vi "列表消息json处理.vi"(6 "error in (no error)":errorcluster caption="错误输入（无错误）", 7 "json input":string) -> (0 "error out":errorcluster caption="错误输出", 1 "top_stories":T1(array[cluster]), 2 "stories":T1(array[cluster]), 3 "date":string)   [LabVIEW 2012]
uses:
  <vilib>/addons/JSON API/JSON Value/JSON Value.lvclass
  <vilib>/addons/JSON API/JSON Value/Set from JSON string.vi
  <vilib>/addons/JSON API/Get Polymorphic/JSON GetSet.lvlib
  <vilib>/addons/JSON API/JSON Scalar/JSON Scalar.lvclass
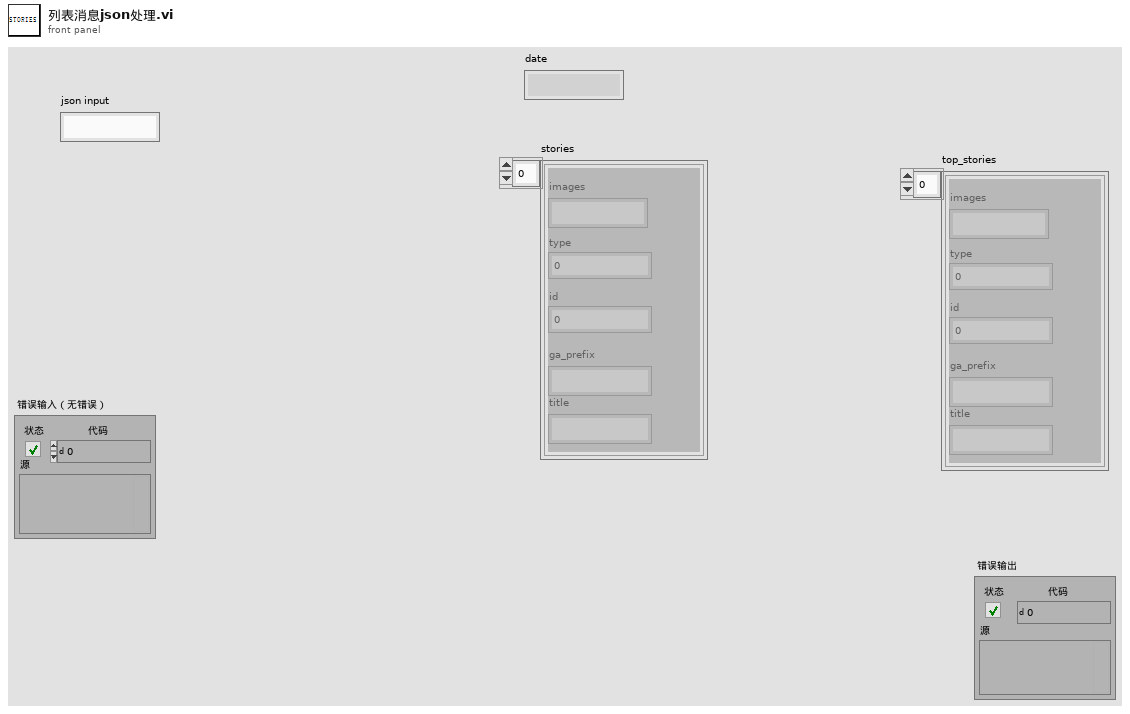
[diagram p1: front panel]
types:
  T1 = cluster{"images":string, "type":i32, "id":i64, "ga_prefix":string, "title":string}[]
  T2 = cluster{"LabVIEW Text":string, "Number":i32, "Number":i32, "LabVIEW Text":string, "LabVIEW Text":string}
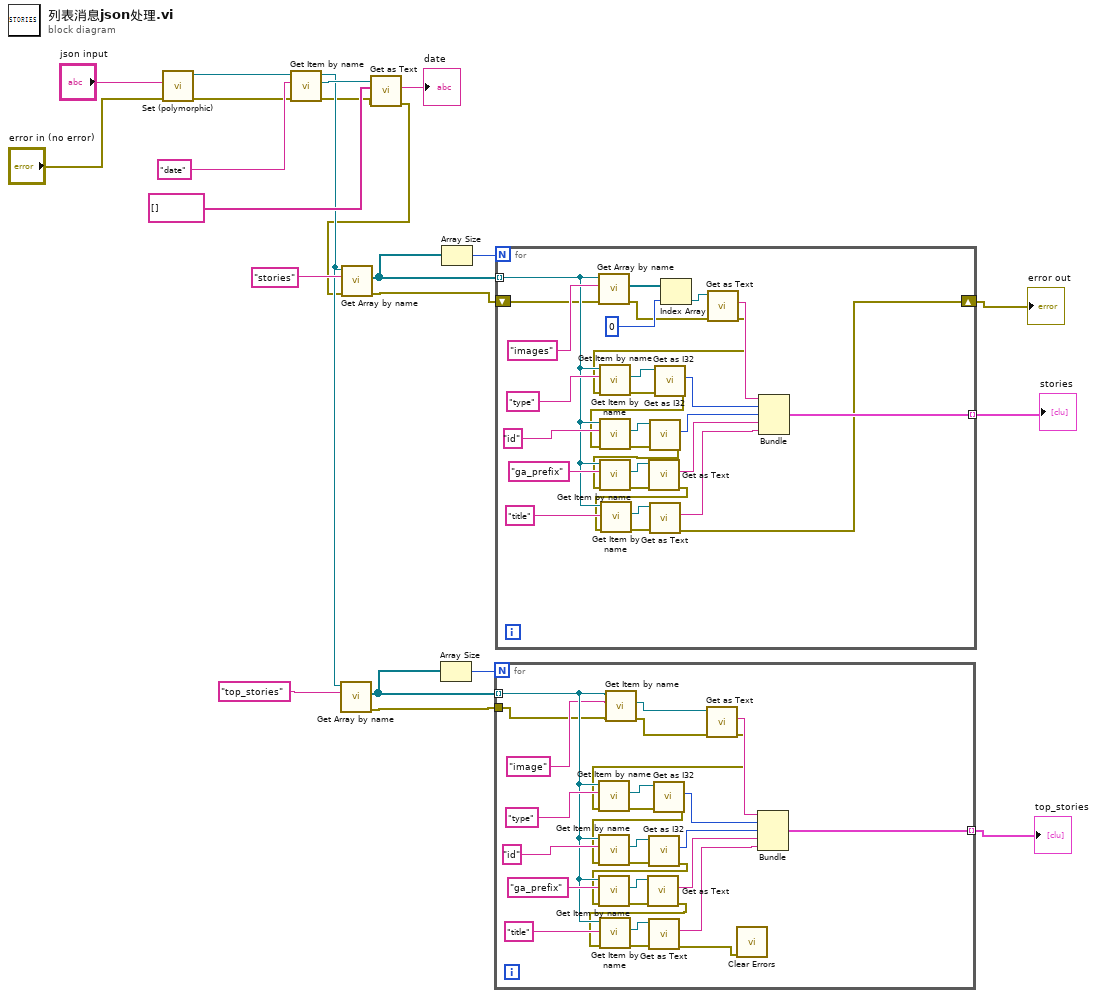
[diagram p0: block diagram]
diagram:
  n1 = call-poly <vilib>:"Set (polymorphic).vi"("error in (no error)"="error in (no error)", "JSON stream"="json input") -> ("error out"=w20:errorcluster, "JSON Value out"=w22:refnum<class "JSON Value.lvclass">)  [unwired: 7 in, 1 out]
  n2 = call-dynamic "Get Item by name.vi"("error in (no error)"=w20, "name"="date", "JSON Value In"=w22) -> ("error out"=w3:errorcluster, "Value"=w19:refnum<class "JSON Value.lvclass">, "JSON Value Out"=w6:refnum<class "JSON Value.lvclass">)  [unwired: 5 in, 1 out]
  n3 = call <vilib>:"Get Array by name.vi"("name"="top_stories", "JSON Value In"=w6) -> ("error out"=w7:errorcluster, "Array"=w8:refnum<class "JSON Value.lvclass">[])  [unwired: 6 in, 2 out]
  n4 = call <vilib>:"Get as Text.vi"("error in (no error)"=w3, "Name Array"=string[] [], "JSON Scalar in"=w19) -> ("error out"=w2:errorcluster, "LabVIEW Text"=→"date":string)  [unwired: 6 in, 1 out]
  n5 = call <vilib>:"Get Array by name.vi"("error in (no error)"=w2, "name"="stories", "JSON Value In"=w6) -> ("error out"=w12:errorcluster, "Array"=w13:refnum<class "JSON Value.lvclass">[])  [unwired: 5 in, 2 out]
  n6 = Array Size(array=w8) -> (size(s)=w9:i32)
  n7 = Array Size(array=w13) -> (size(s)=w14:i32)
  n8 = for {
    N: w9 -> [_]
    tunnel: w8 -> [w32] mode=indexing
    tunnel: w7 -> [w30]
    tunnel: [w33] -> w5 mode=indexing
    n9 = call-dynamic "Get Item by name.vi"("error in (no error)"=w30, "name"="image", "JSON Value In"=w32) -> ("error out"=w28:errorcluster, "Value"=w29:refnum<class "JSON Value.lvclass">)  [unwired: 5 in, 2 out]
    n10 = call <vilib>:"Get as Text.vi"("error in (no error)"=w28, "JSON Scalar in"=w29) -> ("error out"=w27:errorcluster, "LabVIEW Text"=w38:string)  [unwired: 7 in, 1 out]
    n11 = call-dynamic "Get Item by name.vi"("error in (no error)"=w27, "name"="type", "JSON Value In"=w32) -> ("error out"=w45:errorcluster, "Value"=w49:refnum<class "JSON Value.lvclass">)  [unwired: 5 in, 2 out]
    n12 = call <vilib>:"Get as I32.vi"("error in (no error)"=w45, "JSON Scalar in"=w49) -> ("error out"=w26:errorcluster, "Number"=w37:i32)  [unwired: 7 in, 1 out]
    n13 = call-dynamic "Get Item by name.vi"("error in (no error)"=w26, "name"="id", "JSON Value In"=w32) -> ("error out"=w46:errorcluster, "Value"=w47:refnum<class "JSON Value.lvclass">)  [unwired: 5 in, 2 out]
    n14 = call <vilib>:"Get as I32.vi"("error in (no error)"=w46, "JSON Scalar in"=w47) -> ("error out"=w25:errorcluster, "Number"=w36:i32)  [unwired: 7 in, 1 out]
    n15 = call-dynamic "Get Item by name.vi"("error in (no error)"=w25, "name"="ga_prefix", "JSON Value In"=w32) -> ("error out"=w42:errorcluster, "Value"=w43:refnum<class "JSON Value.lvclass">)  [unwired: 5 in, 2 out]
    n16 = call <vilib>:"Get as Text.vi"("error in (no error)"=w42, "JSON Scalar in"=w43) -> ("error out"=w24:errorcluster, "LabVIEW Text"=w35:string)  [unwired: 7 in, 1 out]
    n17 = call-dynamic "Get Item by name.vi"("error in (no error)"=w24, "name"="title", "JSON Value In"=w32) -> ("error out"=w39:errorcluster, "Value"=w40:refnum<class "JSON Value.lvclass">)  [unwired: 5 in, 2 out]
    n18 = call <vilib>:"Get as Text.vi"("error in (no error)"=w39, "JSON Scalar in"=w40) -> ("error out"=w23:errorcluster, "LabVIEW Text"=w34:string)  [unwired: 7 in, 1 out]
    n19 = call <vilib>:"Clear Errors.vi"("error in (no error)"=w23) -> ()  [unwired: 6 in, 1 out]
    n20 = Bundle("LabVIEW Text"=w38, "Number"=w37, "Number"=w36, "LabVIEW Text"=w35, "LabVIEW Text"=w34) -> (w33:T2)  [unwired: 1 in]
  }
  "top_stories" <- w5
  n21 = for {
    N: w14 -> [_]
    tunnel: w13 -> [w66] mode=indexing
    tunnel: [w56] -> w11 mode=indexing
    shift-right: [w51] -> w1
    shift-left: w12 -> [w65]
    n22 = call <vilib>:"Get Array by name.vi"("error in (no error)"=w65, "name"="images", "JSON Value In"=w66) -> ("error out"=w70:errorcluster, "Array"=w79:refnum<class "JSON Value.lvclass">[])  [unwired: 5 in, 2 out]
    n23 = Index Array(array=w79, index=0) -> (element=w77:refnum<class "JSON Value.lvclass">)
    n24 = call <vilib>:"Get as Text.vi"("error in (no error)"=w70, "JSON Scalar in"=w77) -> ("error out"=w55:errorcluster, "LabVIEW Text"=w61:string)  [unwired: 7 in, 1 out]
    n25 = call-dynamic "Get Item by name.vi"("error in (no error)"=w55, "name"="type", "JSON Value In"=w66) -> ("error out"=w71:errorcluster, "Value"=w75:refnum<class "JSON Value.lvclass">)  [unwired: 5 in, 2 out]
    n26 = call <vilib>:"Get as I32.vi"("error in (no error)"=w71, "JSON Scalar in"=w75) -> ("error out"=w54:errorcluster, "Number"=w60:i32)  [unwired: 7 in, 1 out]
    n27 = call-dynamic "Get Item by name.vi"("error in (no error)"=w54, "name"="id", "JSON Value In"=w66) -> ("error out"=w72:errorcluster, "Value"=w73:refnum<class "JSON Value.lvclass">)  [unwired: 5 in, 2 out]
    n28 = call <vilib>:"Get as I32.vi"("error in (no error)"=w72, "JSON Scalar in"=w73) -> ("error out"=w53:errorcluster, "Number"=w59:i32)  [unwired: 7 in, 1 out]
    n29 = call-dynamic "Get Item by name.vi"("error in (no error)"=w53, "name"="ga_prefix", "JSON Value In"=w66) -> ("error out"=w67:errorcluster, "Value"=w68:refnum<class "JSON Value.lvclass">)  [unwired: 5 in, 2 out]
    n30 = call <vilib>:"Get as Text.vi"("error in (no error)"=w67, "JSON Scalar in"=w68) -> ("error out"=w52:errorcluster, "LabVIEW Text"=w58:string)  [unwired: 7 in, 1 out]
    n31 = call-dynamic "Get Item by name.vi"("error in (no error)"=w52, "name"="title", "JSON Value In"=w66) -> ("error out"=w62:errorcluster, "Value"=w63:refnum<class "JSON Value.lvclass">)  [unwired: 5 in, 2 out]
    n32 = call <vilib>:"Get as Text.vi"("error in (no error)"=w62, "JSON Scalar in"=w63) -> ("error out"=w51:errorcluster, "LabVIEW Text"=w57:string)  [unwired: 7 in, 1 out]
    n33 = Bundle("LabVIEW Text"=w61, "Number"=w60, "Number"=w59, "LabVIEW Text"=w58, "LabVIEW Text"=w57) -> (w56:T2)  [unwired: 1 in]
  }
  "stories" <- w11
  "error out" <- w1
